vi "Suffix Duplicated VI--constant.vi"() -> (3 "Suffix Duplicated VI":string)   [LabVIEW 2026]
doc: "This constant represents a string added to the end of file names to avoid conflicts during project creation."
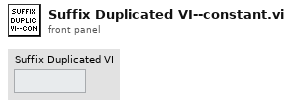
[diagram p1: front panel]
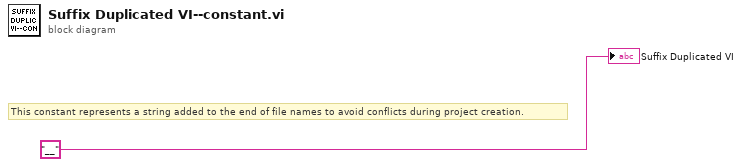
[diagram p0: block diagram]
diagram:
  # "This constant represents a string added to the end of file names to avoid conflicts during project creation."
  "Suffix Duplicated VI" <- "__" ("Suffix Duplicated VI")
